vi "query Call Processing Status.vi"(8 "error in (no error)":errorcluster, 11 "Anritsu Call Box_Implement in":refnum<class "Anritsu Call Box_Implement.lvclass">) -> (0 "error out":errorcluster, 2 "Call Processing Status":T1, 3 "Anritsu Call Box_Implement out":refnum<class "Anritsu Call Box_Implement.lvclass">)   [LabVIEW 2023, in "ANRITSU Call Box.lvlib" / "Anritsu Call Box_Implement.lvclass"]
doc: "Call Processing Status는 NR / LTE 동일."
uses:
  Anritsu Call Box_Implement.lvclass
  Type Definition/Call Processing Status Enum.ctl
  Anritsu Call Box_Implement.lvclass/Anritsu Call Box_Implement.ctl
  NR/NR.lvclass
  LTE/LTE.lvclass
  ANRITSU Call Box.lvlib
  D:/Project/IST027_FCC Main EIRP and RSE Measurement/Source Code/Module/ANRITSU Call Box/Implement Class/Anritsu Call Box_Implement/Anritsu Call Box_Implement.lvclass
  D:/Project/IST027_FCC Main EIRP and RSE Measurement/Source Code/Module/ANRITSU Call Box/Interface Class/Anritsu Call Box.lvclass
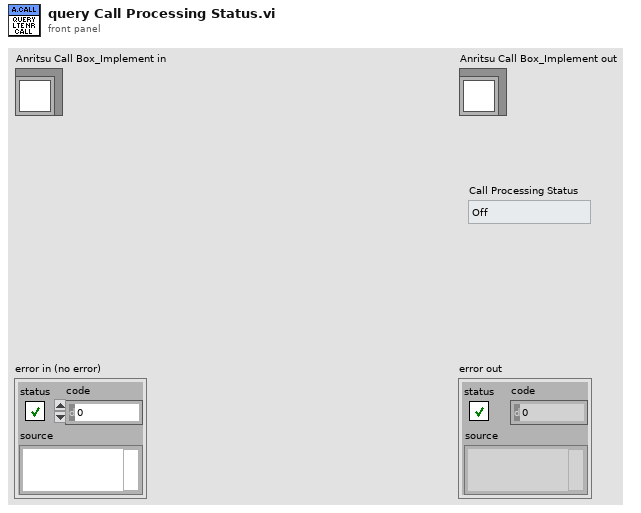
[diagram p1: front panel]
types:
  T1 = typedef "ANRITSU Call Box.lvlib/Call Processing Status Enum.ctl" = enum16{"Off", "Idle", "Idle (Regist)", "Registration", "UE Origination", "NW Origination", "Connected", "SCG Adding", "Connected (NSA)", "SCG Release", "Undefined1", "Undefined2", "Undefined3", "Handover", "NW Release", "UE Release", "Detach", "Setup", "Redirection"}
  T2 = typedef "ANRITSU Call Box.lvlib/Call Device - Protocol Type Selector.ctl" = enum16{"8000A - NR", "8000A - LTE", "882xC - LTE"}
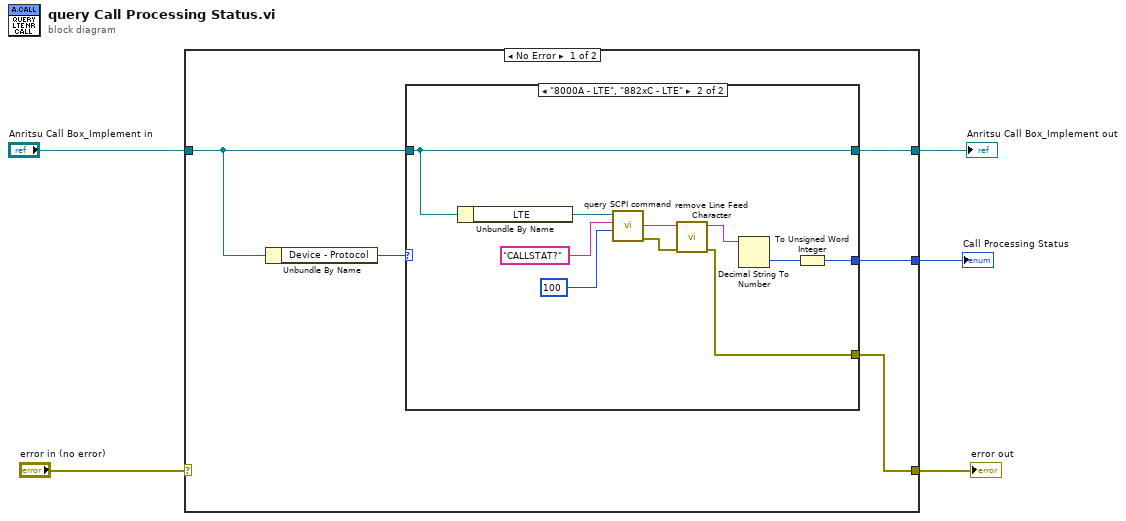
[diagram p0: block diagram]
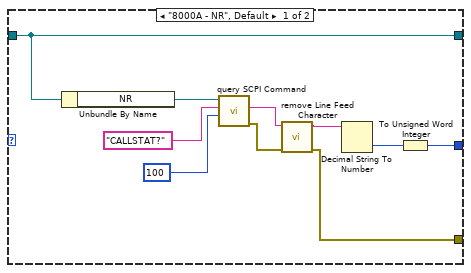
[diagram p2: hidden frame]
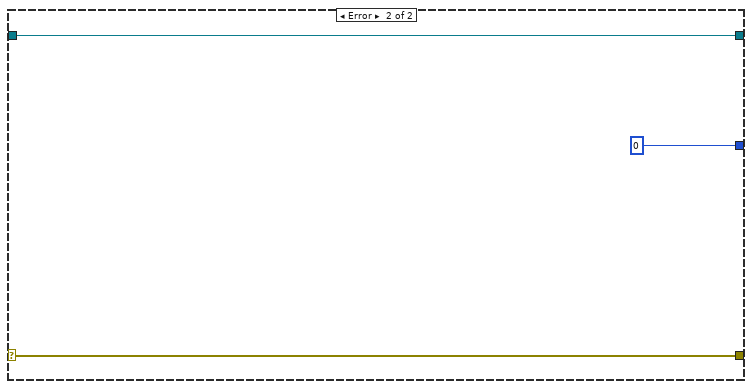
[diagram p3: hidden frame]
diagram:
  n1 = case shown="No Error" "error in (no error)" {
    selector: "error in (no error)" -> [_ w32]
    tunnel: "Anritsu Call Box_Implement in" -> [w9 w33]
    tunnel: [w7 w33] -> w3
    tunnel: [w6 w32] -> w2
    tunnel: [w8 u16 0] -> w1
    frame No Error {
      n2 = Unbundle By Name(w9) -> ("Device - Protocol"=w10:T2)
      n3 = case shown="\"8000A - LTE\", \"882xC - LTE\"" w10 {
        tunnel: w9 -> [w15 w21]
        tunnel: [w16 w29] -> w8
        tunnel: [w15 w21] -> w7
        tunnel: [w11 w22] -> w6
        frame "8000A - NR", Default {
          n4 = Unbundle By Name(w15) -> ("NR"=w20:refnum<class "NR.lvclass">)
          n5 = call "query SCPI Command.vi"("Read Buffer Length"=u32 100 ("byte count"), "SCPI Command"="CALLSTAT?" ("write buffer"), "NR in"=w20) -> ("error out"=w13:errorcluster, "Read Buffer String"=w14:string)  [unwired: 6 in, 1 out]
          n6 = call "remove Line Feed Character.vi"("error in"=w13, "Query String"=w14) -> ("error out"=w11:errorcluster, "Line Feed Removed String"=w12:string)  [unwired: 8 in]
          n7 = Decimal String To Number(string=w12) -> (number=w17:i32)  [unwired: 2 in, 1 out]
          n8 = To Unsigned Word Integer(number=w17) -> (unsigned 16bit integer=w16:u16)
        }
        frame "8000A - LTE", "882xC - LTE" {
          n9 = Unbundle By Name(w21) -> ("LTE"=w28:refnum<class "LTE.lvclass">)
          n10 = call "query SCPI command.vi"("Read Buffer Length"=u32 100 ("byte count"), "SCPI Command"="CALLSTAT?" ("write buffer"), "LTE in"=w28) -> ("error out"=w24:errorcluster, "Read Buffer String"=w25:string)  [unwired: 6 in, 1 out]
          n11 = call "remove Line Feed Character.vi"("error in"=w24, "Query String"=w25) -> ("error out"=w22:errorcluster, "Line Feed Removed String"=w23:string)  [unwired: 8 in]
          n12 = Decimal String To Number(string=w23) -> (number=w30:i32)  [unwired: 2 in, 1 out]
          n13 = To Unsigned Word Integer(number=w30) -> (unsigned 16bit integer=w29:u16)
        }
      }
    }
    frame Error {
    }
  }
  "error out" <- w2
  "Anritsu Call Box_Implement out" <- w3
  "Call Processing Status" <- w1
